vi "query NR UL_DL Center Channel Number.vi"(8 "error in (no error)":errorcluster, 9 "Direction":T2, 10 "Selected CC Argements":T1, 11 "Anritsu Call Box_Implement in":refnum<class "Anritsu Call Box_Implement.lvclass">) -> (0 "error out":errorcluster, 2 "Center Channel Number":u32, 3 "Anritsu Call Box_Implement out":refnum<class "Anritsu Call Box_Implement.lvclass">)   [LabVIEW 2023, in "ANRITSU Call Box.lvlib" / "Anritsu Call Box_Implement.lvclass"]
uses:
  Anritsu Call Box_Implement.lvclass
  Anritsu Call Box_Implement.lvclass/Anritsu Call Box_Implement.ctl
  NR/NR.lvclass
  Type Definition/Uplink Downlink Enum.ctl
  ANRITSU Call Box.lvlib
  Type Definition/NR Selected CC Type Arguments.ctl
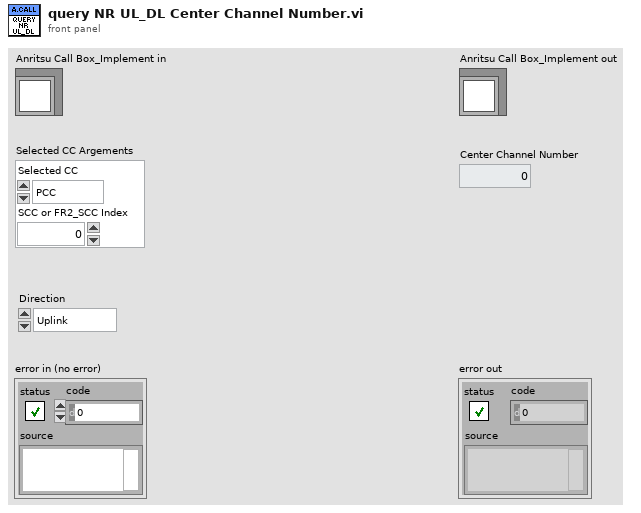
[diagram p1: front panel]
types:
  T1 = typedef "ANRITSU Call Box.lvlib/NR Selected CC Type Arguments.ctl" = cluster{"Selected CC":enum16{"PCC", "SCC", "FR2_PCC", "FR2_SCC"}, "SCC or FR2_SCC Index":u32}
  T2 = typedef "ANRITSU Call Box.lvlib/Uplink Downlink Enum.ctl" = enum16{"Uplink", "Downlink"}
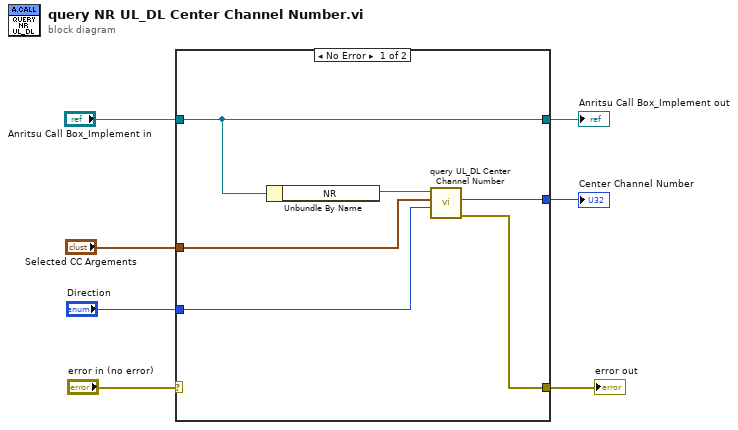
[diagram p0: block diagram]
diagram:
  n1 = case shown="No Error" "error in (no error)" {
    selector: "error in (no error)" -> [_ w14]
    tunnel: "Anritsu Call Box_Implement in" -> [w13 w15]
    tunnel: [w13 w15] -> w6
    tunnel: [w8 w14] -> w4
    tunnel: "Selected CC Argements" -> [w11 _]
    tunnel: [w9 _] -> w1
    tunnel: "Direction" -> [w10 _]
    frame No Error {
      n2 = Unbundle By Name(w13) -> ("NR"=w12:refnum<class "NR.lvclass">)
      n3 = call "query UL_DL Center Channel Number.vi"("Direction"=w10, "Selected CC Argements"=w11, "NR in"=w12) -> ("error out"=w8:errorcluster, "Center Channel Number"=w9:u32)  [unwired: 6 in, 1 out]
    }
    frame Error {
    }
  }
  "error out" <- w4
  "Anritsu Call Box_Implement out" <- w6
  "Center Channel Number" <- w1
